vi "TwoButtonDialogAsync.vi"(0 "message":string, 2 "File dialog event":T1, 5 "T button name (\"OK\")":string, 7 "F button name (\"Cancel\")":string, 11 "error in":errorcluster) -> (15 "error out":errorcluster)   [LabVIEW 2025]
uses:
  FileDialogEvent.ctl
  FileDialogResult.ctl
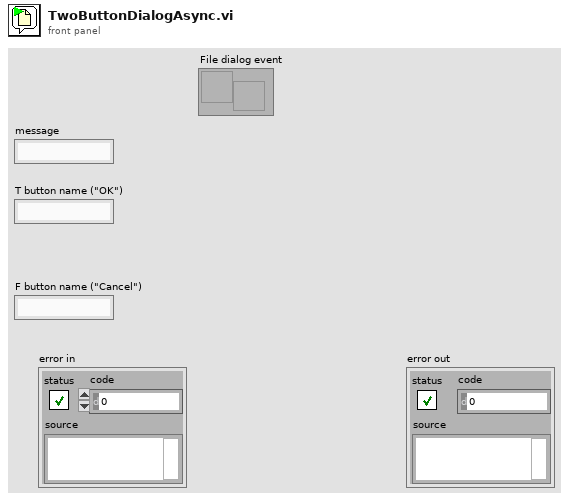
[diagram p1: front panel]
types:
  T1 = typedef "FileDialogEvent.ctl" = refnum<user-event>
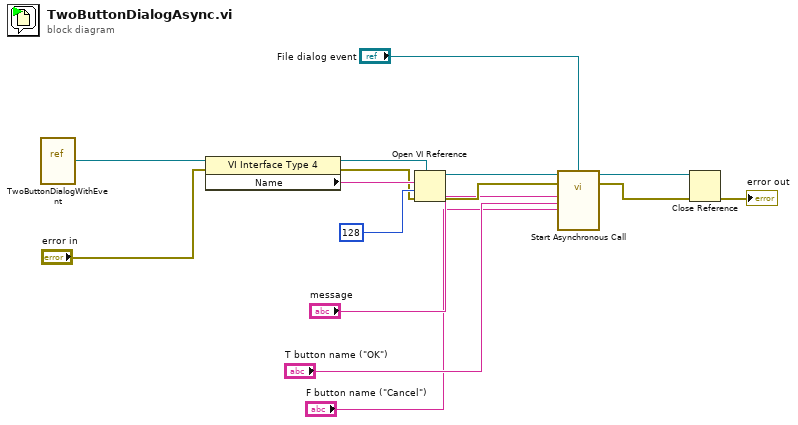
[diagram p0: block diagram]
diagram:
  n1 = vi-ref "TwoButtonDialogWithEvent.vi"() -> (w11:refnum<vi>)
  n2 = property class="VI Interface Type 4"(reference=w11, error in="error in") -> (reference out=w4:refnum<vi>, error out=w9:errorcluster, "Name"=w15:string)
  n3 = Open VI Reference(type specifier VI Refnum (for type only)=w4, vi path=w15, options=128, error in (no error)=w9) -> (vi reference=w10:refnum<vi>, error out=w7:errorcluster)  [unwired: 2 in]
  n4 = call-by-ref "Start Asynchronous Call"(reference=w10, error in=w7, "message"="message", "File dialog event"="File dialog event", "T button name (\"OK\")"="T button name (\"OK\")", "F button name (\"Cancel\")"="F button name (\"Cancel\")") -> (reference out=w14:refnum<vi>, error out=w13:errorcluster)  [unwired: 12 in]
  n5 = Close Reference(reference=w14, error in (no error)=w13) -> (error out=→"error out":errorcluster)
